vi "test Add-Find-Remove.vi"(8 "error in":errorcluster, 11 "TestCase in":refnum<class "Scripting.lvclass">) -> (0 "error out":errorcluster, 3 "TestCase out":refnum<class "Scripting.lvclass">)   [LabVIEW 2020, in "Scripting.lvclass"]
uses:
  Scripting.lvclass
  <vilib>/NI VeriStand/Custom Device API/Custom Device Item Ref.ctl
  Shared/Direction.ctl
  Shared/SDI.ctl
  Scripting.lvclass/Scripting.ctl
  Shared/Transfer Type.ctl
  <vilib>/addons/_JKI Toolkits/VI Tester/TestCase.llb/TestCase.lvclass
  <vilib>/NI VeriStand/Custom Device API/Custom Device API.lvlib
  Scripting/AIM/AIM ARINC 429 Scripting.lvlib
  Shared/Transfer Speed.ctl
  C:/Program Files (x86)/National Instruments/LabVIEW 2020/vi.lib/addons/_JKI Toolkits/VI Tester/TestCase.llb/TestCase.lvclass
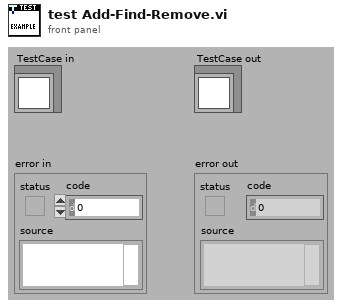
[diagram p1: front panel]
types:
  T1 = typedef "Transfer Speed.ctl" = enum16{"LO (12.5 kb/s)", "HI (100 kb/s)"}
  T2 = typedef "Direction.ctl" = enum16{"Rx", "Tx"}
  T3 = typedef "Custom Device API.lvlib/Custom Device Item Ref.ctl" = u64
  T4 = typedef "Transfer Type.ctl" = enum16{"Scheduled", "Acyclic", "Block", "Strobe"}
  T5 = typedef "SDI.ctl" = i32
  T6 = typedef "Custom Device API.lvlib/Custom Device Item Info.ctl" = cluster{"Name":string, "Is Channel":bool, "GUID":string, "Is Waveform":bool}
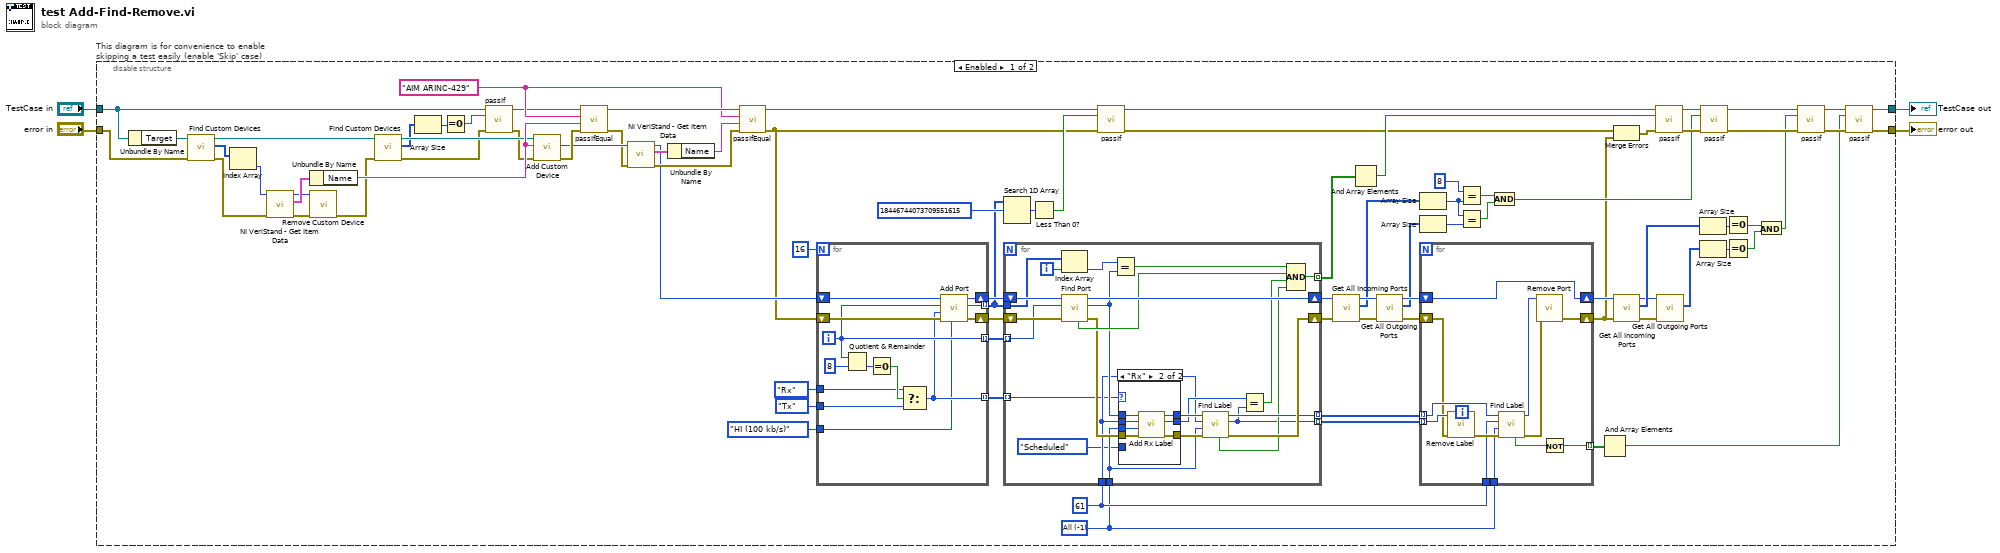
[diagram p0: block diagram]
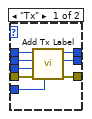
[diagram p2: hidden frame]
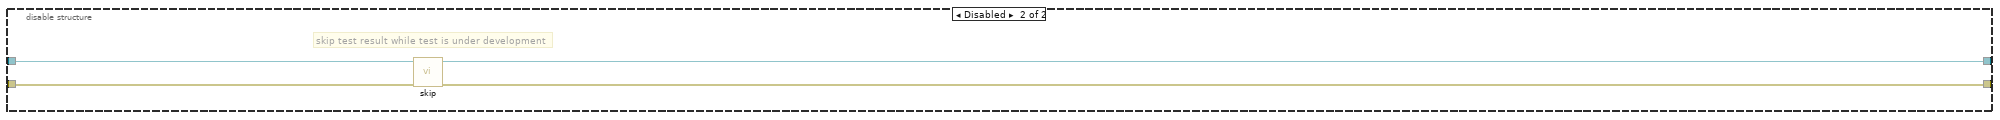
[diagram p3: hidden frame]
diagram:
  n1 = disable-structure "This diagram is for convenience to enable skipping a test easily (enable 'Skip' case)" shown="Enabled" {
    disable-tunnel: "TestCase in" -> [w70 w158]
    disable-tunnel: [w8 w156] -> w1
    disable-tunnel: [w9 w157] -> w3
    disable-tunnel: "error in" -> [w88 w155]
    frame Enabled {
      w14 = u32 61 ("label value")
      w13 = T5 -1 items=["All"=-1, "0 (b00)"=0, "1 (b01)"=1, "2 (b10)"=2, "3 (b11)"=3] ("SDI value")
      w76 = "AIM ARINC-429" ("string")
      n2 = Unbundle By Name(w70) -> ("Target"=w90:refnum<k24>)
      n3 = call "Find Custom Devices.vi"("error in"=w88, "target in"=w90) -> ("error out"=w85:errorcluster, "AIM ARINC 429 custom devices"=w87:u64[], "target out"=w73:refnum<k24>)  [unwired: 7 in]
      n4 = Index Array(array=w87) -> (element=w86:u64)  [unwired: 1 in]
      n5 = call <vilib>:"NI VeriStand - Get Item Data.vi"("error in (no error)"=w85, "Item Ref in"=w86) -> ("error out"=w74:errorcluster, "Item Info"=w84:T6, "Item Ref out"=w75:T3)  [unwired: 6 in, 1 out]
      n6 = Unbundle By Name(w84) -> ("Name"=w78:string)
      n7 = call "Remove Custom Device.vi"("error in"=w74, "AIM ARINC 429 custom device"=w75) -> ("error out"=w71:errorcluster)  [unwired: 9 in]
      n8 = call "Find Custom Devices.vi"("error in"=w71, "target in"=w73) -> ("error out"=w69:errorcluster, "AIM ARINC 429 custom devices"=w66:u64[], "target out"=w72:refnum<k24>)  [unwired: 7 in]
      n9 = Array Size(array=w66) -> (size(s)=w65:i32)
      n10 = Equal To 0?(x=w65) -> (x = 0?=w64:bool)
      n11 = call-dynamic "passIf.vi"("error in (no error)"=w69, "pass"=w64, "TestCase in"=w70) -> ("error out"=w67:errorcluster, "TestCase out"=w68:refnum<class "Scripting.lvclass">)  [unwired: 7 in]
      n12 = call "Add Custom Device.vi"("error in"=w67, "name"=w78, "target in"=w72) -> ("error out"=w83:errorcluster, "AIM ARINC 429 custom device"=w82:T3)  [unwired: 6 in, 1 out]
      n13 = call-dynamic "passIfEqual.vi"("error in (no error)"=w83, "y"=w78, "x"=w76, "TestCase in"=w68) -> ("error out"=w81:errorcluster, "TestCase out"=w89:refnum<class "Scripting.lvclass">)  [unwired: 6 in]
      n14 = call <vilib>:"NI VeriStand - Get Item Data.vi"("error in (no error)"=w81, "Item Ref in"=w82) -> ("error out"=w79:errorcluster, "Item Info"=w80:T6, "Item Ref out"=w63:T3)  [unwired: 6 in, 1 out]
      n15 = Unbundle By Name(w80) -> ("Name"=w77:string)
      n16 = call-dynamic "passIfEqual.vi"("error in (no error)"=w79, "y"=w77, "x"=w76, "TestCase in"=w89) -> ("error out"=w19:errorcluster, "TestCase out"=w22:refnum<class "Scripting.lvclass">)  [unwired: 6 in]
      n17 = for {
        N: 16 -> [_]
        shift-right: [w150] -> w62
        shift-left: w63 -> [w154]
        tunnel: [w149] -> w56 mode=indexing
        shift-right: [w147] -> w61
        shift-left: w19 -> [w148]
        tunnel: [w146] -> w60 mode=indexing
        tunnel: Direction."Rx" ("direction") -> [w145]
        tunnel: Direction."Tx" ("direction") -> [w144]
        tunnel: [w143] -> w6 mode=indexing
        tunnel: Transfer_Speed."HI (100 kb/s)" ("speed") -> [w142]
        i -> [w146]
        n18 = Quotient & Remainder(x=w146, y=8) -> (floor(x/y)=w152:i32)  [unwired: 1 out]
        n19 = Equal To 0?(x=w152) -> (x = 0?=w151:bool)
        n20 = Select(t=w145, s=w151, f=w144) -> (s? t:f=w143:T2)
        n21 = call "Add Port.vi"("speed"=w142, "error in"=w148, "direction"=w143, "port number"=w146, "AIM ARINC 429 custom device in"=w154) -> ("error out"=w147:errorcluster, "port"=w149:T3, "AIM ARINC 429 custom device out"=w150:T3)  [unwired: 4 in]
      }
      n22 = Search 1D Array(1D array=w56, element=T3 18446744073709551615 ("custom device ref out")) -> (index of element=w23:i32)  [unwired: 1 in]
      n23 = for {
        shift-right: [w125] -> w53
        shift-left: w62 -> [w126]
        tunnel: w60 -> [w123] mode=indexing
        tunnel: w56 -> [w120]
        shift-right: [w112] -> w52
        shift-left: w61 -> [w124]
        tunnel: [w111] -> w58 mode=indexing
        tunnel: [w117] -> w42 mode=indexing
        tunnel: [w107] -> w15 mode=indexing
        tunnel: w13 -> [w106]
        tunnel: w14 -> [w105]
        tunnel: w6 -> [w103] mode=indexing
        i -> [w122]
        n24 = Index Array(array=w120, index=w122) -> (element=w121:T3)
        n25 = call "Find Port.vi"("error in"=w124, "port number"=w123, "AIM ARINC 429 custom device in"=w126) -> ("error out"=w113:errorcluster, "port"=w114:T3, "AIM ARINC 429 custom device out"=w125:T3, "found?"=w118:bool)  [unwired: 5 in]
        n26 = Equal?(x=w121, y=w114) -> (x = y?=w119:bool)
        n27 = case shown="\"Rx\"" w103 {
          tunnel: [w134 w141] -> w116
          tunnel: [w133 w140] -> w115
          tunnel: w114 -> [w132 w139]
          tunnel: w113 -> [w131 w138]
          tunnel: [w130 w137] -> w110
          tunnel: w106 -> [w129 w136]
          tunnel: w105 -> [w128 w135]
          tunnel: Transfer_Type."Scheduled" ("transfer type") -> [w127 _]
          frame "Tx" {
            n28 = call "Add Tx Label.vi"("transfer type"=w127, "error in"=w131, "SDI value"=w129, "label value"=w128, "port in"=w132) -> ("error out"=w134:errorcluster, "label"=w130:T3, "port out"=w133:T3)  [unwired: 4 in]
          }
          frame "Rx" {
            n29 = call "Add Rx Label.vi"("error in"=w138, "SDI value"=w136, "label value"=w135, "port in"=w139) -> ("error out"=w141:errorcluster, "label"=w137:T3, "port out"=w140:T3)  [unwired: 5 in]
          }
        }
        n30 = call "Find Label.vi"("error in"=w116, "SDI value"=w106, "label value"=w105, "port in"=w115) -> ("error out"=w112:errorcluster, "label"=w107:T3, "port out"=w111:T3, "found?"=w109:bool)  [unwired: 4 in]
        n31 = Equal?(x=w110, y=w107) -> (x = y?=w108:bool)
        n32 = Compound Arithmetic op=AND(w119, w118, w108, w109) -> (w117:bool)
      }
      n33 = Less Than 0?(x=w23) -> (x < 0?=w20:bool)
      n34 = call-dynamic "passIf.vi"("error in (no error)"=w19, "pass"=w20, "TestCase in"=w22) -> ("error out"=w18:errorcluster, "TestCase out"=w21:refnum<class "Scripting.lvclass">)  [unwired: 7 in]
      n35 = call "Get All Incoming Ports.vi"("error in"=w52, "AIM ARINC 429 custom device in"=w53) -> ("error out"=w54:errorcluster, "incoming ports"=w49:T3[], "AIM ARINC 429 custom device out"=w55:T3)  [unwired: 7 in]
      n36 = And Array Elements(Boolean array=w42) -> (logical AND=w39:bool)
      n37 = call "Get All Outgoing Ports.vi"("error in"=w54, "AIM ARINC 429 custom device in"=w55) -> ("error out"=w50:errorcluster, "outgoing ports"=w48:T3[], "AIM ARINC 429 custom device out"=w51:T3)  [unwired: 7 in]
      n38 = Array Size(array=w49) -> (size(s)=w46:i32)
      n39 = Array Size(array=w48) -> (size(s)=w47:i32)
      n40 = for {
        shift-right: [w102] -> w29
        shift-left: w51 -> [w102]
        shift-right: [w101] -> w17
        shift-left: w50 -> [w98]
        tunnel: w58 -> [w99] mode=indexing
        tunnel: w15 -> [w100] mode=indexing
        tunnel: w14 -> [w96]
        tunnel: w13 -> [w95]
        tunnel: [w91] -> w12 mode=indexing
        n41 = call "Remove Label.vi"("error in"=w98, "label"=w100) -> ("error out"=w97:errorcluster)  [unwired: 9 in]
        n42 = call "Find Label.vi"("error in"=w97, "SDI value"=w95, "label value"=w96, "port in"=w99) -> ("error out"=w94:errorcluster, "port out"=w93:T3, "found?"=w92:bool)  [unwired: 4 in, 1 out]
        n43 = call "Remove Port.vi"("error in"=w94, "port"=w93) -> ("error out"=w101:errorcluster)  [unwired: 9 in]
        n44 = Not(x=w92) -> (.not. x?=w91:bool)
      }
      n45 = Equal?(x=8, y=w46) -> (x = y?=w44:bool)
      n46 = Equal?(x=w46, y=w47) -> (x = y?=w43:bool)
      n47 = And(x=w44, y=w43) -> (x .and. y?=w38:bool)
      n48 = And Array Elements(Boolean array=w12) -> (logical AND=w7:bool)
      n49 = Merge Errors(w18, w17) -> (w16:errorcluster)
      n50 = call "Get All Incoming Ports.vi"("error in"=w17, "AIM ARINC 429 custom device in"=w29) -> ("error out"=w31:errorcluster, "incoming ports"=w32:T3[], "AIM ARINC 429 custom device out"=w30:T3)  [unwired: 7 in]
      n51 = call-dynamic "passIf.vi"("error in (no error)"=w16, "pass"=w39, "TestCase in"=w21) -> ("error out"=w40:errorcluster, "TestCase out"=w41:refnum<class "Scripting.lvclass">)  [unwired: 7 in]
      n52 = call "Get All Outgoing Ports.vi"("error in"=w31, "AIM ARINC 429 custom device in"=w30) -> ("outgoing ports"=w33:T3[])  [unwired: 7 in, 2 out]
      n53 = Array Size(array=w32) -> (size(s)=w35:i32)
      n54 = Array Size(array=w33) -> (size(s)=w34:i32)
      n55 = call-dynamic "passIf.vi"("error in (no error)"=w40, "pass"=w38, "TestCase in"=w41) -> ("error out"=w27:errorcluster, "TestCase out"=w28:refnum<class "Scripting.lvclass">)  [unwired: 7 in]
      n56 = Equal To 0?(x=w35) -> (x = 0?=w36:bool)
      n57 = Equal To 0?(x=w34) -> (x = 0?=w37:bool)
      n58 = And(x=w36, y=w37) -> (x .and. y?=w26:bool)
      n59 = call-dynamic "passIf.vi"("error in (no error)"=w27, "pass"=w26, "TestCase in"=w28) -> ("error out"=w11:errorcluster, "TestCase out"=w10:refnum<class "Scripting.lvclass">)  [unwired: 7 in]
      n60 = call-dynamic "passIf.vi"("error in (no error)"=w11, "pass"=w7, "TestCase in"=w10) -> ("error out"=w9:errorcluster, "TestCase out"=w8:refnum<class "Scripting.lvclass">)  [unwired: 7 in]
    }
    frame Disabled {
      # "skip test result while test is under development"
      n61 = call <vilib>:"skip.vi"("error in (no error)"=w155, "TestCase in"=w158) -> ("error out"=w157:errorcluster, "TestCase out"=w156:refnum<class "Scripting.lvclass">)  [unwired: 8 in]
    }
  }
  "error out" <- w3
  "TestCase out" <- w1
